vi "Door_Open.vi"(0 "State":T1={"Tick"=0, "Phase"=0, "PhaseTicks"=0, "Level"=1, "Room"=0, "X10"=0, "Y10"=0, "VY10"=0, "Mode"=0, "Facing"=0, "Run"=0, "Vert"=0, "StandY"=0, "EntryX10"=0, "EntryY10"=0, "EntryMode"=0, "Lives"=4, "Score"=0, "NextLife"=10000, "KeyR"=0, "KeyB"=0, "KeyY"=0, "Torch"=FALSE, "FloorPhase"=0, "Dead"=FALSE, "LevelStart"=FALSE, "Quit"=FALSE, "Sound"=0, "Seed"=12345, "DemoStep"=0, "Tiles"=[], "World"=[], "Enemies"=[], "Highscores"=[], "Name"=[0, 0, 0], "Cursor"=0}, 11 "error in":errorcluster) -> (4 "State out":T1={"Tick"=0, "Phase"=0, "PhaseTicks"=0, "Level"=1, "Room"=0, "X10"=0, "Y10"=0, "VY10"=0, "Mode"=0, "Facing"=0, "Run"=0, "Vert"=0, "StandY"=0, "EntryX10"=0, "EntryY10"=0, "EntryMode"=0, "Lives"=4, "Score"=0, "NextLife"=10000, "KeyR"=0, "KeyB"=0, "KeyY"=0, "Torch"=FALSE, "FloorPhase"=0, "Dead"=FALSE, "LevelStart"=FALSE, "Quit"=FALSE, "Sound"=0, "Seed"=12345, "DemoStep"=0, "Tiles"=[], "World"=[], "Enemies"=[], "Highscores"=[], "Name"=[0, 0, 0], "Cursor"=0}, 6 "Opened":bool, 15 "error out":errorcluster)   [LabVIEW 2020, in "GH_Engine.lvlib"]
doc: "Opens the door Claude touches (in the direction he faces) when he has a key of its colour: the key is used up, all tiles of that door (one column, up to 3 tiles above and below) become empty, +100 points, door sound."
uses:
  GH_Engine.lvlib
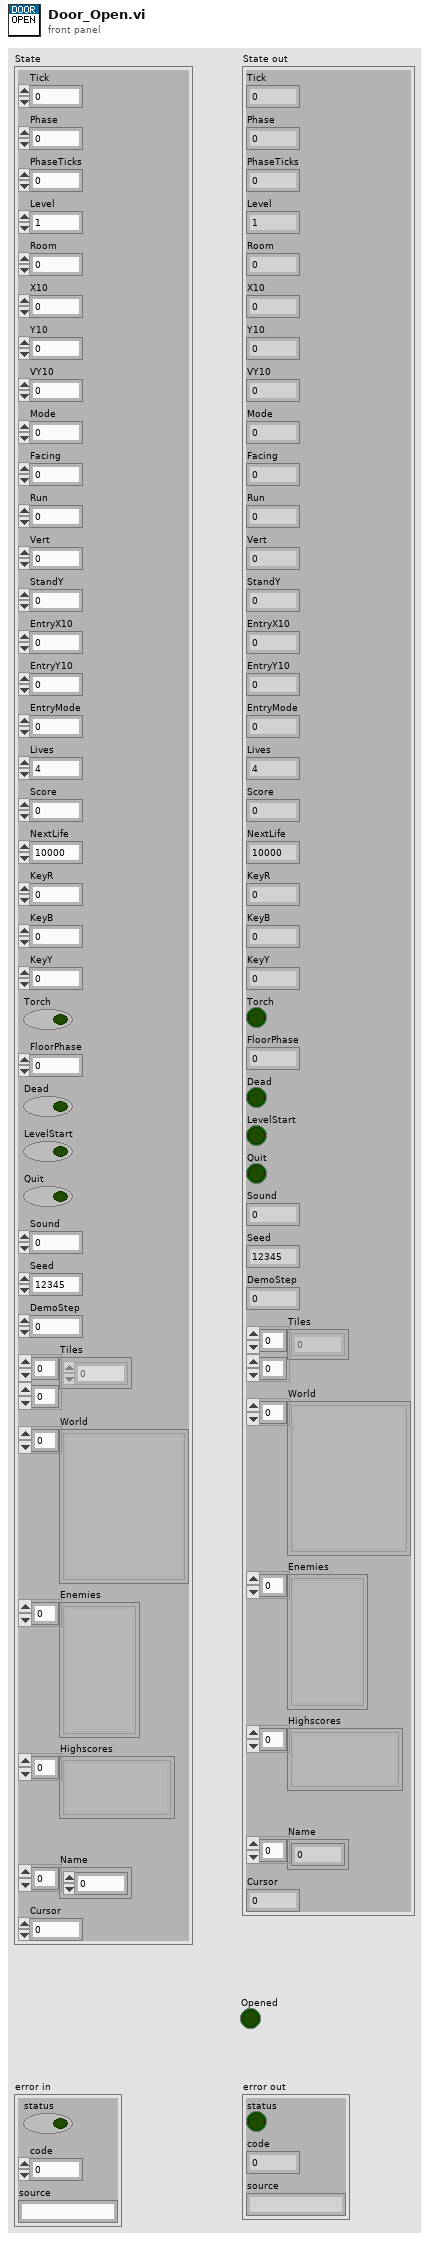
[diagram p1: front panel]
types:
  T1 = cluster{"Tick":u32, "Phase":i32, "PhaseTicks":i32, "Level":i32, "Room":i32, "X10":i32, "Y10":i32, "VY10":i32, "Mode":i32, "Facing":i32, "Run":i32, "Vert":i32, "StandY":i32, "EntryX10":i32, "EntryY10":i32, "EntryMode":i32, "Lives":i32, "Score":i32, "NextLife":i32, "KeyR":i32, "KeyB":i32, "KeyY":i32, "Torch":bool, "FloorPhase":i32, "Dead":bool, "LevelStart":bool, "Quit":bool, "Sound":i32, "Seed":u32, "DemoStep":i32, "Tiles":u8[][], "World":cluster{"ID":string, "Depth":i32, "Column":i32, "Tiles":u8[][]}[], "Enemies":cluster{"Kind":i32, "X10":i32, "Y10":i32, "Dir":i32, "Mode":i32}[], "Highscores":cluster{"Score":i32, "Name":string}[], "Name":i32[], "Cursor":i32}
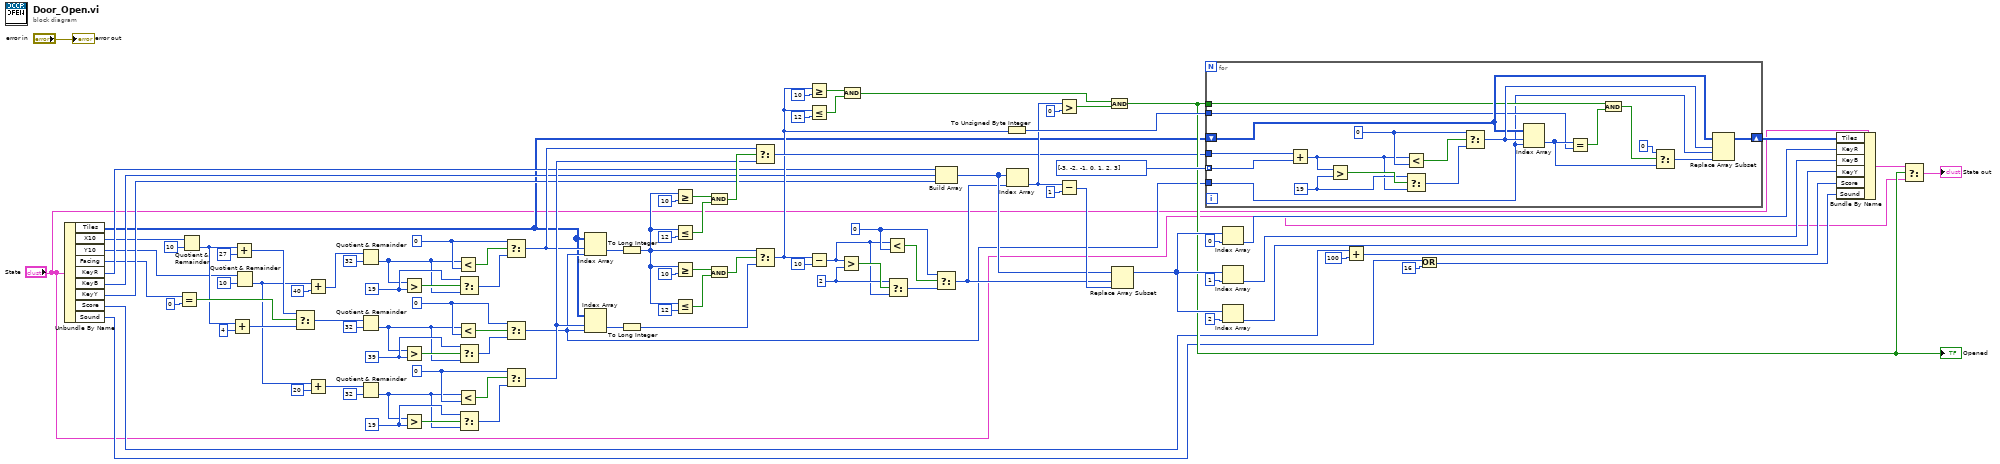
[diagram p0: block diagram]
diagram:
  w70 = 2
  w69 = 0
  w46 = 19
  w45 = 0
  w36 = 19
  w35 = 0
  w26 = 39
  w25 = 0
  n1 = Unbundle By Name("State") -> ("Tiles"=w3:u8[][], "X10"=w4:i32, "Y10"=w5:i32, "Facing"=w6:i32, "KeyR"=w7:i32, "KeyB"=w8:i32, "KeyY"=w9:i32, "Score"=w10:i32, "Sound"=w11:i32)
  n2 = Equal?(x=w6, y=0) -> (x = y?=w17:bool)
  n3 = Quotient & Remainder(x=w4, y=10) -> (floor(x/y)=w13:i32)  [unwired: 1 out]
  n4 = Add(x=w13, y=4) -> (x+y=w21:i32)
  n5 = Add(x=w13, y=27) -> (x+y=w19:i32)
  n6 = Quotient & Remainder(x=w5, y=10) -> (floor(x/y)=w15:i32)  [unwired: 1 out]
  n7 = Select(t=w19, s=w17, f=w21) -> (s? t:f=w22:i32)
  n8 = Add(x=w15, y=40) -> (x+y=w32:i32)
  n9 = Add(x=w15, y=20) -> (x+y=w42:i32)
  n10 = Quotient & Remainder(x=w32, y=32) -> (floor(x/y)=w34:i32)  [unwired: 1 out]
  n11 = Quotient & Remainder(x=w22, y=32) -> (floor(x/y)=w24:i32)  [unwired: 1 out]
  n12 = Quotient & Remainder(x=w42, y=32) -> (floor(x/y)=w44:i32)  [unwired: 1 out]
  n13 = Greater?(x=w34, y=w36) -> (0:w38:bool)
  n14 = Greater?(x=w24, y=w26) -> (0:w28:bool)
  n15 = Greater?(x=w44, y=w46) -> (0:w48:bool)
  n16 = Less?(x=w34, y=w35) -> (x < y?=w37:bool)
  n17 = Less?(x=w24, y=w25) -> (x < y?=w27:bool)
  n18 = Less?(x=w44, y=w45) -> (x < y?=w47:bool)
  n19 = Select(t=w36, s=w38, f=w34) -> (s? t:f=w39:i32)
  n20 = Select(t=w26, s=w28, f=w24) -> (s? t:f=w29:i32)
  n21 = Select(t=w46, s=w48, f=w44) -> (s? t:f=w49:i32)
  n22 = Select(t=w35, s=w37, f=w39) -> (s? t:f=w40:i32)
  n23 = Select(t=w25, s=w27, f=w29) -> (s? t:f=w30:i32)
  n24 = Select(t=w45, s=w47, f=w49) -> (s? t:f=w50:i32)
  n25 = Index Array(array=w3, index (row)=w40, index (col)=w30) -> (element=w51:u8)
  n26 = Index Array(array=w3, index (row)=w50, index (col)=w30) -> (element=w53:u8)
  n27 = To Long Integer(number=w51) -> (32bit integer=w52:i32)
  n28 = To Long Integer(number=w53) -> (32bit integer=w54:i32)
  n29 = Greater Or Equal?(x=w52, y=10) -> (x >= y?=w62:bool)
  n30 = Less Or Equal?(x=w52, y=12) -> (x <= y?=w64:bool)
  n31 = Greater Or Equal?(x=w52, y=10) -> (x >= y?=w56:bool)
  n32 = Less Or Equal?(x=w52, y=12) -> (x <= y?=w58:bool)
  n33 = And(x=w62, y=w64) -> (x .and. y?=w65:bool)
  n34 = And(x=w56, y=w58) -> (x .and. y?=w59:bool)
  n35 = Select(t=w40, s=w65, f=w50) -> (s? t:f=w66:i32)
  n36 = Select(t=w52, s=w59, f=w54) -> (s? t:f=w60:i32)
  n37 = Greater Or Equal?(x=w60, y=10) -> (x >= y?=w78:bool)
  n38 = Less Or Equal?(x=w60, y=12) -> (x <= y?=w80:bool)
  n39 = Subtract(x=w60, y=10) -> (x-y=w68:i32)
  n40 = Greater?(x=w68, y=w70) -> (0:w72:bool)
  n41 = And(x=w78, y=w80) -> (x .and. y?=w81:bool)
  n42 = Less?(x=w68, y=w69) -> (x < y?=w71:bool)
  n43 = Select(t=w70, s=w72, f=w68) -> (s? t:f=w73:i32)
  n44 = Build Array(w7, w8, w9) -> (w75:i32[])
  n45 = Select(t=w69, s=w71, f=w73) -> (s? t:f=w74:i32)
  n46 = To Unsigned Byte Integer(number=w60) -> (unsigned 8bit integer=w86:u8)
  n47 = Index Array(array=w75, index=w74) -> (element=w76:i32)
  n48 = Greater?(x=w76, y=0) -> (0:w83:bool)
  n49 = Subtract(x=w76, y=1) -> (x-y=w89:i32)
  n50 = And(x=w81, y=w83) -> (x .and. y?=w84:bool)
  "Opened" <- w84
  n51 = Replace Array Subset(array=w75, new element=w89, index=w74) -> (w90:i32[])
  n52 = for {
    tunnel: i32[] [-3, -2, -1, 0, 1, 2, 3] ("Rows around") -> [w103] mode=indexing
    shift-right: [w109] -> w87
    shift-left: w3 -> [w108]
    tunnel: w30 -> [w105]
    tunnel: w66 -> [w104]
    tunnel: w86 -> [w106]
    tunnel: w84 -> [w107]
    w112 = 19
    w111 = 0
    n53 = Add(x=w104, y=w103) -> (x+y=w110:i32)
    n54 = Greater?(x=w110, y=w112) -> (0:w114:bool)
    n55 = Less?(x=w110, y=w111) -> (x < y?=w113:bool)
    n56 = Select(t=w112, s=w114, f=w110) -> (s? t:f=w115:i32)
    n57 = Select(t=w111, s=w113, f=w115) -> (s? t:f=w116:i32)
    n58 = Index Array(array=w108, index (row)=w116, index (col)=w105) -> (element=w117:u8)
    n59 = Equal?(x=w117, y=w106) -> (x = y?=w118:bool)
    n60 = And(x=w107, y=w118) -> (x .and. y?=w119:bool)
    n61 = Select(t=u8 0, s=w119, f=w117) -> (s? t:f=w121:u8)
    n62 = Replace Array Subset(array=w108, new element=w121, index (row)=w116, index (col)=w105) -> (w109:u8[][])
  }
  n63 = Index Array(array=w90, index=0) -> (element=w92:i32)
  n64 = Index Array(array=w90, index=1) -> (element=w94:i32)
  n65 = Index Array(array=w90, index=2) -> (element=w96:i32)
  n66 = Add(x=w10, y=100) -> (x+y=w98:i32)
  n67 = Or(x=w11, y=16) -> (x .or. y?=w100:i32)
  n68 = Bundle By Name(cluster="State", "Tiles"=w87, "KeyR"=w92, "KeyB"=w94, "KeyY"=w96, "Score"=w98, "Sound"=w100) -> (w101:T1)
  n69 = Select(t=w101, s=w84, f="State") -> (s? t:f=→"State out":T1)
  "error out" <- "error in"
